vi "G-Open-Uart.vi"(7 "Mask":T1=48 items=["I/O接收缓冲区"=16, "I/O传输缓冲区"=32, "I/O接收和传输缓冲区"=48], 8 "error in (no error)":errorcluster caption="错误输入（无错误）", 9 "大小(4096)":u32=100000, 10 "数组":T2(array[cluster]), 11 "G-Uart-Class 输入":refnum<class "G-Uart-Class.lvclass">) -> (0 "error out":errorcluster caption="错误输出", 2 "数组 2":refnum<visa-resource-name>[](array[refnum]), 3 "G-Uart-Class 输出":refnum<class "G-Uart-Class.lvclass">)   [LabVIEW 2025, in "G-Uart-Class.lvclass"]
uses:
  G-Uart-Class.lvclass
  <vilib>/Instr/_visa.llb/VISA Set IO Buffer Mask.ctl
  <vilib>/Instr/_visa.llb/VISA Configure Serial Port (Instr).vi
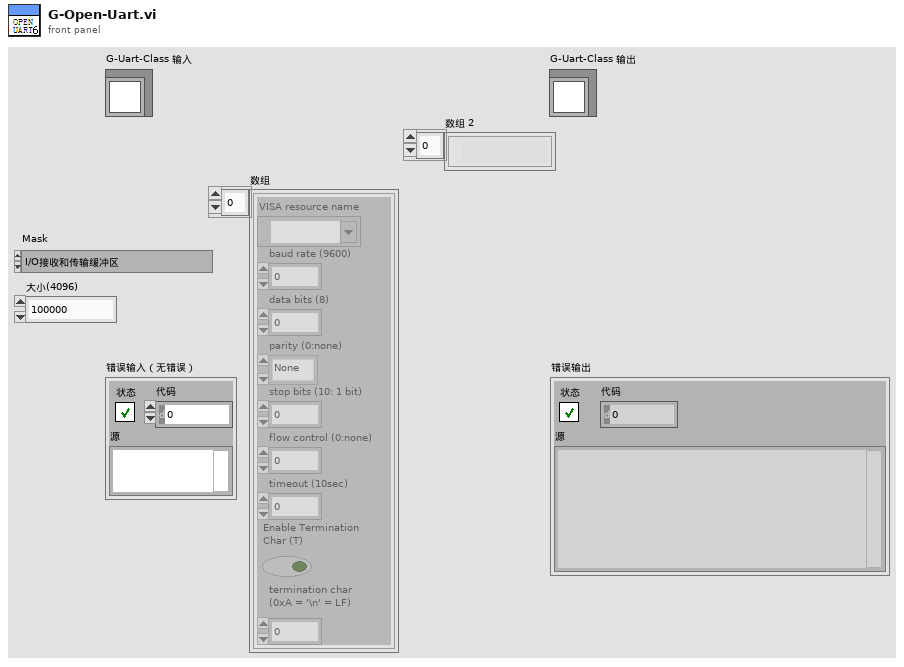
[diagram p1: front panel]
types:
  T1 = typedef "VISA Set IO Buffer Mask.ctl" = u16
  T2 = cluster{"VISA resource name":refnum<visa-resource-name>, "baud rate (9600)":u32, "data bits (8)":u16, "parity (0:none)":enum16{"None", "Odd", "Even", "Mark", "Space"}, "stop bits (10: 1 bit)":u16, "flow control (0:none)":u16, "timeout (10sec)":u32, "Enable Termination\nChar (T)":bool, "termination char\n(0xA = '\\n' = LF) ":u8}[]
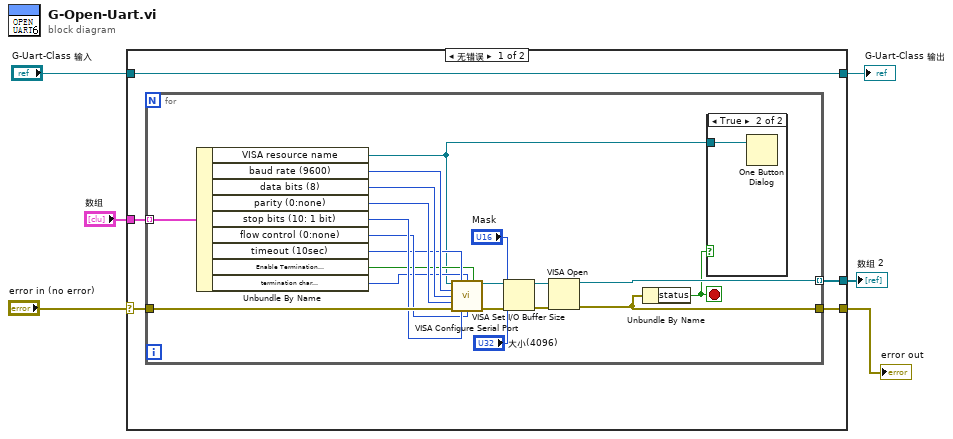
[diagram p0: block diagram]
diagram:
  n1 = case shown="无错误" "error in (no error)" {
    selector: "error in (no error)" -> [w9 w34]
    tunnel: [w8 w34] -> w5
    tunnel: [w11 w33] -> w3
    tunnel: "G-Uart-Class 输入" -> [w11 w33]
    tunnel: "数组" -> [w10 _]
    tunnel: [w7 _] -> w1
    frame No Error {
      n2 = for {
        tunnel: w10 -> [w31] mode=indexing
        tunnel: w9 -> [w30]
        tunnel: [w21] -> w7 mode=indexing
        tunnel: [w19] -> w8
        stop <- w18 stop-if-true
        n3 = Unbundle By Name(w31) -> ("VISA resource name"=w20:refnum<visa-resource-name>, "baud rate (9600)"=w29:u32, "data bits (8)"=w28:u16, "parity (0:none)"=w27:enum16{"None", "Odd", "Even", "Mark", "Space"}, "stop bits (10: 1 bit)"=w26:u16, "flow control (0:none)"=w25:u16, "timeout (10sec)"=w24:u32, "Enable Termination\nChar (T)"=w22:bool, "termination char\n(0xA = '\\n' = LF)"=w23:u8)
        n4 = call-poly "VISA Configure Serial Port"("VISA resource name"=w20, "timeout (10sec)"=w24, "termination char\n(0xA = '\\n' = LF)"=w23, "Enable Termination\nChar (T)"=w22, "baud rate (9600)"=w29, "data bits (8)"=w28, "parity (0:none)"=w27, "error in (no error)"=w30, "stop bits (10: 1 bit)"=w26, "flow control (0:none)"=w25) -> ("VISA resource name out"=w16:refnum<visa-resource-name>, "error out"=w17:errorcluster)  [unwired: 4 in]
        n5 = VISA Set I/O Buffer Size(VISA resource name=w16, mask (16)="Mask", size (4096)="大小(4096)", error in (no error)=w17) -> (VISA resource name out=w12:refnum<visa-resource-name>, error out=w13:errorcluster)
        n6 = VISA Open(error in (no error)=w13, VISA resource name=w12) -> (VISA resource name=w21:refnum<visa-resource-name>, error out=w19:errorcluster)  [unwired: 3 in]
        n7 = Unbundle By Name(w19) -> ("status"=w18:bool)
        n8 = case shown="True" w18 {
          tunnel: w20 -> [_ w32]
          frame False {
          }
          frame True {
            n9 = One Button Dialog(message=w32) -> ()  [unwired: 1 in, 1 out]
          }
        }
      }
    }
    frame Error {
    }
  }
  "error out" <- w5
  "G-Uart-Class 输出" <- w3
  "数组 2" <- w1
